vi "RemoteVI Check Splitters Message.vi"() -> (4 "labels":string[](array[string]), 6 "expected":string[](array[string]), 8 "actual":string[](array[string]), 10 "failures":i32)   [LabVIEW 2020]
doc: "Test support, generated by tests/caraya/build.py from tests/vectors/text.json (splitters) - do not edit. Calls RemoteVI Splitters Message.vi once per vector: the message is compared as the string it is. Outputs, one element per vector: labels (the vector's name), expected (rendered from the vector), actual (the VI's result rendered the same way), and failures, the number of vectors whose expected and actual differ."
uses:
  source/RemoteVI.lvlib
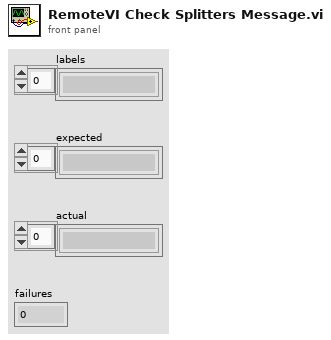
[diagram p1: front panel]
types:
  T1 = cluster{"name":string, "bars":cluster{"x":i32, "y":i32, "w":i32, "h":i32, "vertical":bool, "min":i32, "max":i32}[], "expect":string}[]
  T2 = cluster{"x":i32, "y":i32, "w":i32, "h":i32, "vertical":bool, "min":i32, "max":i32}[]
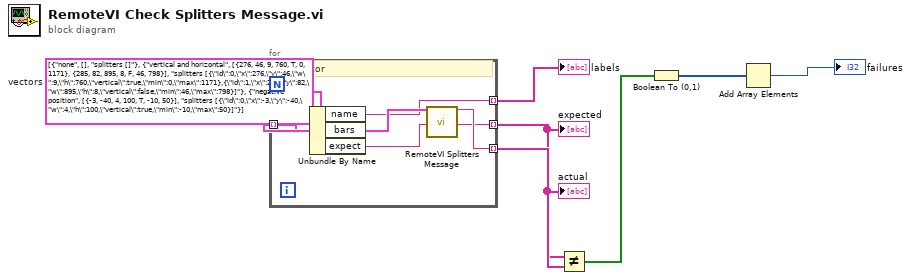
[diagram p0: block diagram]
diagram:
  w1 = T1 [{"name"="none", "bars"=[], "expect"="splitters []"}, {"name"="vertical and horizontal", "bars"=[{"x"=276, "y"=46, "w"=9, "h"=760, "vertical"=TRUE, "min"=0, "max"=1171}, {"x"=285, "y"=82, "w"=895, "h"=8, "vertical"=FALSE, "min"=46, "max"=798}], "expect"="splitters [{\"id\":0,\"x\":276,\"y\":46,\"w\":9,\"h\":760,\"vertical\":true,\"min\":0,\"max\":1171},{\"id\":1,\"x\":285,\"y\":82,\"w\":895,\"h\":8,\"vertical\":false,\"min\":46,\"max\":798}]"}, {"name"="negative position", "bars"=[{"x"=-3, "y"=-40, "w"=4, "h"=100, "vertical"=TRUE, "min"=-10, "max"=50}], "expect"="splitters [{\"id\":0,\"x\":-3,\"y\":-40,\"w\":4,\"h\":100,\"vertical\":true,\"min\":-10,\"max\":50}]"}]  # vectors
  n1 = for {
    tunnel: w1 -> [w8] mode=indexing
    tunnel: [w9] -> w2 mode=indexing
    tunnel: [w11] -> w3 mode=indexing
    tunnel: [w12] -> w4 mode=indexing
    # "One vector"
    n2 = Unbundle By Name(w8) -> ("name"=w9:string, "bars"=w10:T2, "expect"=w11:string)
    n3 = call "RemoteVI Splitters Message.vi"("bars"=w10) -> ("message"=w12:string)  [unwired: 14 in]
  }
  "labels" <- w2
  "expected" <- w3
  "actual" <- w4
  n4 = Not Equal?(x=w3, y=w4) -> (x != y?=w5:bool[])
  n5 = Boolean To (0,1)(Boolean=w5) -> (0, 1=w6:i16[])
  n6 = Add Array Elements(numeric array=w6) -> (sum=→"failures":i16)
